vi "String To Number(U16).vi"(5 "String":string) -> (0 "Numeric(U16)":u16)   [LabVIEW 2017]
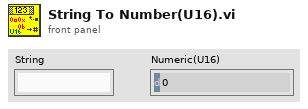
[diagram p1: front panel]
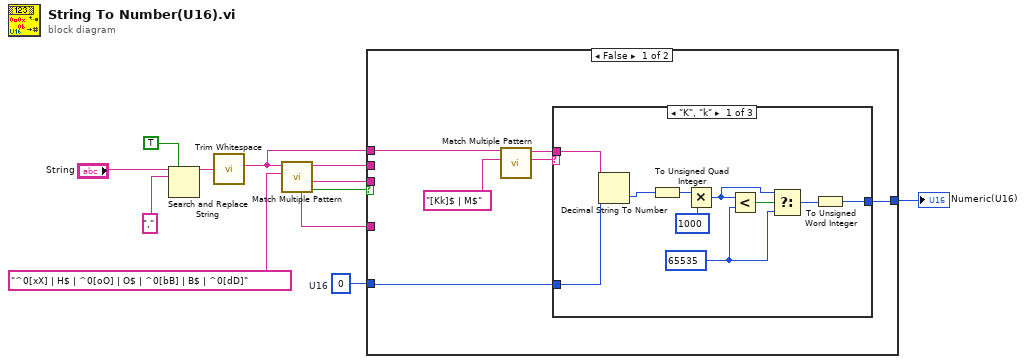
[diagram p0: block diagram]
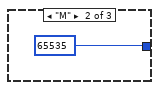
[diagram p2: hidden frame]
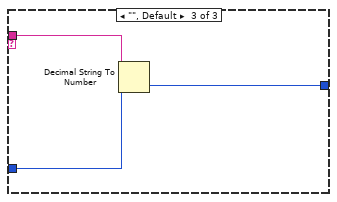
[diagram p3: hidden frame]
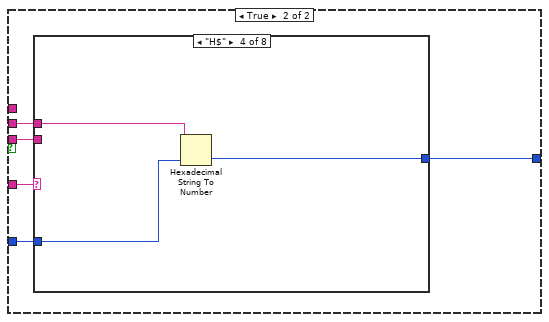
[diagram p4: hidden frame]
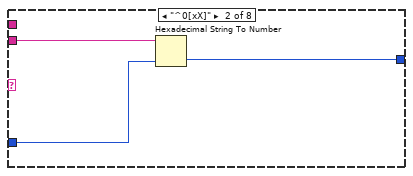
[diagram p6: hidden frame]
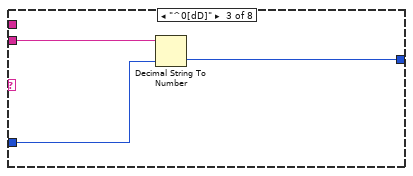
[diagram p7: hidden frame]
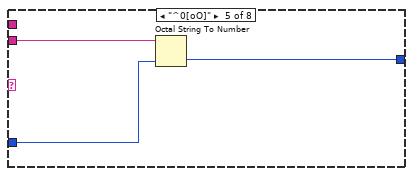
[diagram p8: hidden frame]
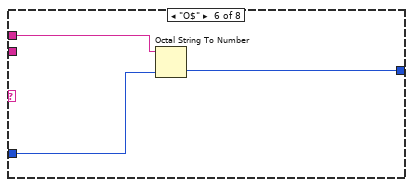
[diagram p9: hidden frame]
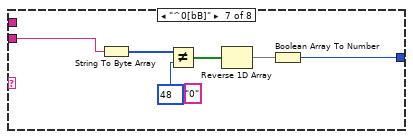
[diagram p10: hidden frame]
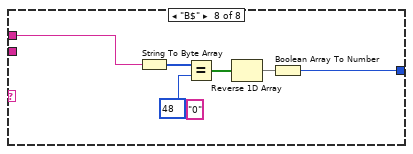
[diagram p11: hidden frame]
diagram:
  w1 = u16 0  # U16
  n1 = Search and Replace String(replace all?=TRUE ("replace all? (F)"), input string="String", search string=",") -> (result string=w9:string)  [unwired: 5 in, 3 out]
  n2 = call <vilib>:"Trim Whitespace.vi"("string"=w9) -> ("trimmed string"=w2:string)  [unwired: 1 in]
  n3 = call "Match Multiple Pattern.vi"("regular expression"="^0[xX] | H$ | ^0[oO] | O$ | ^0[bB] | B$ | ^0[dD]", "string"=w2) -> ("Found?"=w7:bool, "after substring"=w5:string, "before substring"=w4:string, "pattern matched"=w6:string)  [unwired: 5 in, 1 out]
  n4 = case shown="False" w7 {
    tunnel: w6 -> [_ w37]
    tunnel: w5 -> [_ w36]
    tunnel: w4 -> [_ w35]
    tunnel: [w13 w34] -> w3
    tunnel: w2 -> [w14 _]
    tunnel: w1 -> [w15 w33]
    frame False {
      n5 = call "Match Multiple Pattern.vi"("regular expression"="[Kk]$ | M$", "string"=w14) -> ("match substring"=w17:string, "before substring"=w16:string)  [unwired: 5 in, 3 out]
      n6 = case shown="\"K\", \"k\"" w17 {
        tunnel: [w19 u16 65535 ("y") w32] -> w13
        tunnel: w15 -> [w27 _ w31]
        tunnel: w16 -> [w28 _ w30]
        frame "K", "k" {
          w22 = u16 65535 ("y")
          n7 = Decimal String To Number(string=w28, default (0L)=w27) -> (number=w21:u16)  [unwired: 1 in, 1 out]
          n8 = To Unsigned Quad Integer(1:w21) -> (0:w25:u64)
          n9 = Multiply(x=w25, y=u64 1000) -> (x*y=w23:u64)
          n10 = Less?(x=w23, y=w22) -> (x < y?=w24:bool)
          n11 = Select(t=w23, s=w24, f=w22) -> (s? t:f=w20:u64)
          n12 = To Unsigned Word Integer(number=w20) -> (unsigned 16bit integer=w19:u16)
        }
        frame "M" {
        }
        frame "", Default {
          n13 = Decimal String To Number(string=w30, default (0L)=w31) -> (number=w32:u16)  [unwired: 1 in, 1 out]
        }
      }
    }
    frame True {
      n14 = case shown="\"H$\"" w37 {
        tunnel: w36 -> [_ w41 w44 _ w50 _ w58 _]
        tunnel: w35 -> [_ _ _ w46 _ w52 _ w62]
        tunnel: [w38 w40 w43 w47 w49 w53 w59 w65] -> w34
        tunnel: w33 -> [w38 w39 w42 w45 w48 w51 _ _]
        frame Default {
        }
        frame "^0[xX]" {
          n15 = Hexadecimal String To Number(string=w41, default (0uL)=w39) -> (number=w40:u16)  [unwired: 1 in, 1 out]
        }
        frame "^0[dD]" {
          n16 = Decimal String To Number(string=w44, default (0L)=w42) -> (number=w43:u16)  [unwired: 1 in, 1 out]
        }
        frame "H$" {
          n17 = Hexadecimal String To Number(string=w46, default (0uL)=w45) -> (number=w47:u16)  [unwired: 1 in, 1 out]
        }
        frame "^0[oO]" {
          n18 = Octal String To Number(2:w48, 4:w50) -> (0:w49:u16)  [unwired: 1 in, 1 out]
        }
        frame "O$" {
          n19 = Octal String To Number(2:w51, 4:w52) -> (0:w53:u16)  [unwired: 1 in, 1 out]
        }
        frame "^0[bB]" {
          (unwired) "0" ("search string")
          n20 = String To Byte Array(string=w58) -> (unsigned byte array=w57:u8[])
          n21 = Not Equal?(x=w57, y=u8 48) -> (x != y?=w55:bool[])
          n22 = Reverse 1D Array(array=w55) -> (reversed array=w54:bool[])
          n23 = Boolean Array To Number(Boolean array=w54) -> (number=w59:u16)
        }
        frame "B$" {
          (unwired) "0" ("search string")
          n24 = String To Byte Array(string=w62) -> (unsigned byte array=w64:u8[])
          n25 = Equal?(x=w64, y=u8 48) -> (x = y?=w63:bool[])
          n26 = Reverse 1D Array(array=w63) -> (reversed array=w61:bool[])
          n27 = Boolean Array To Number(Boolean array=w61) -> (number=w65:u16)
        }
      }
    }
  }
  "Numeric(U16)" <- w3
